vi "Even or Odd.vi"() -> ()   [LabVIEW 2026]
panel:
  out "Status":string
  in  "Input Number":i64
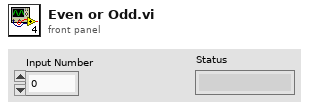
[diagram p1: front panel]
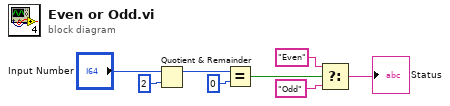
[diagram p0: block diagram]
diagram:
  n1 = Quotient & Remainder(x="Input Number", y=i64 2) -> (x-y*floor(x/y)=w6:i64)  [unwired: 1 out]
  n2 = Equal?(x=w6, y=i64 0) -> (x = y?=w4:bool)
  n3 = Select(t="Even", s=w4, f="Odd") -> (s? t:f=→"Status":string)
